vi "Post-Install Custom Action.vi"(10 "Variant":variant) -> (0 "error out":errorcluster)   [LabVIEW 2015]
panel:
  out "Status":string
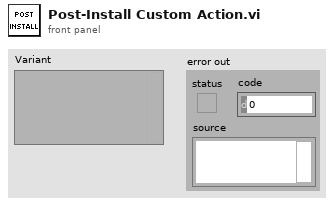
[diagram p1: front panel]
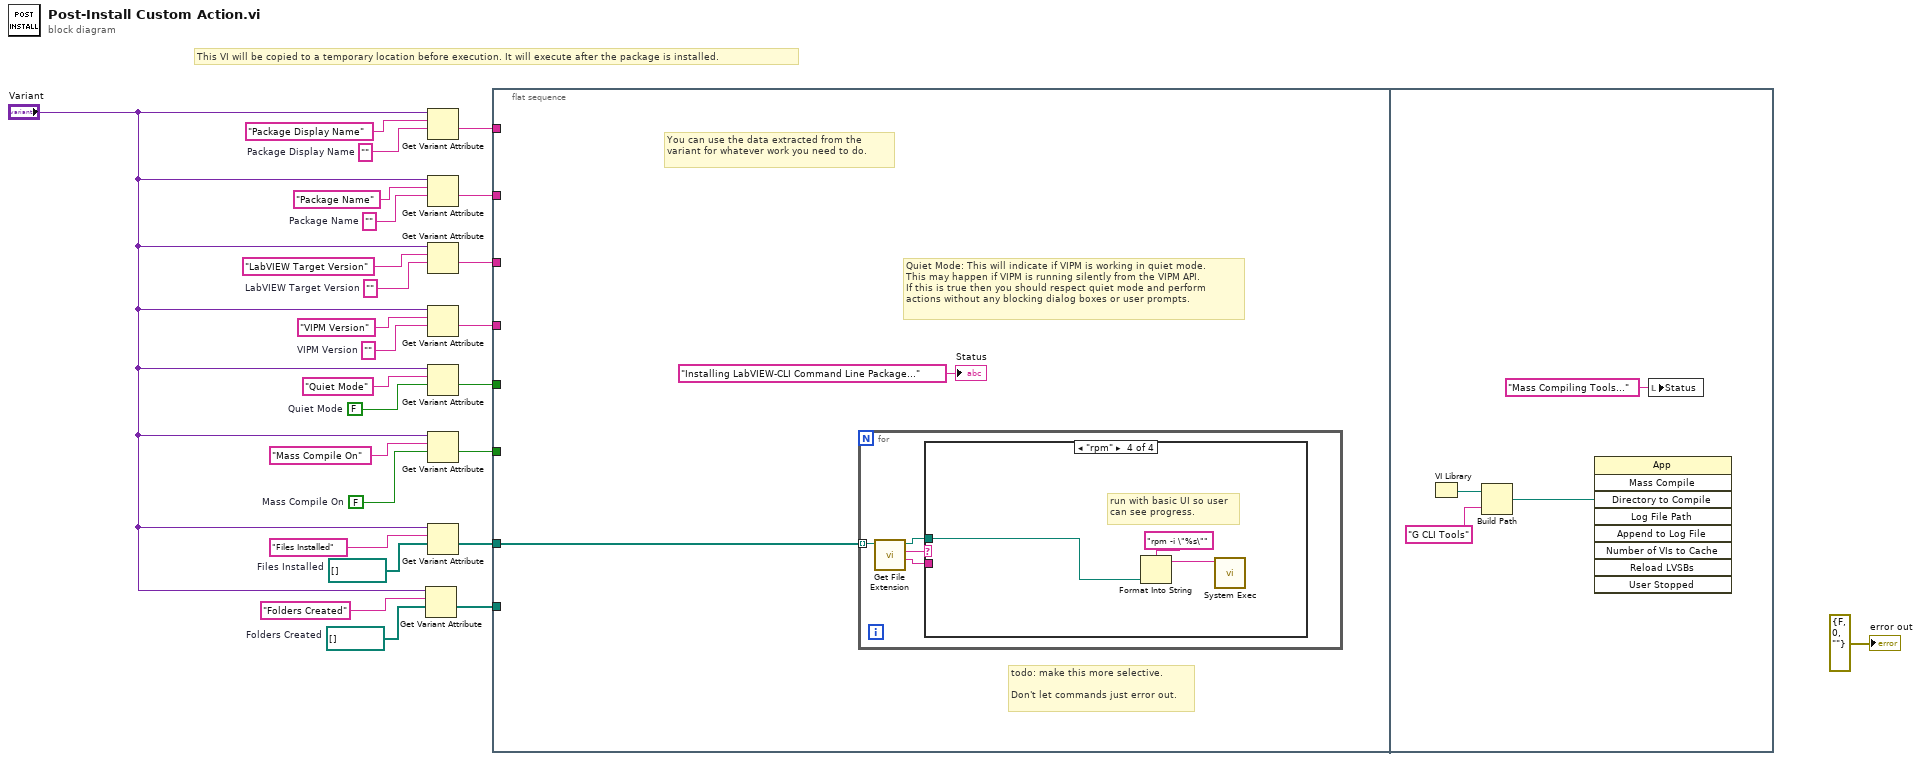
[diagram p0: block diagram]
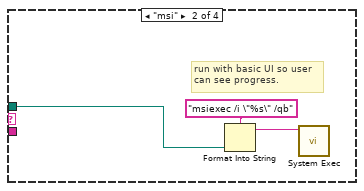
[diagram p3: hidden frame]
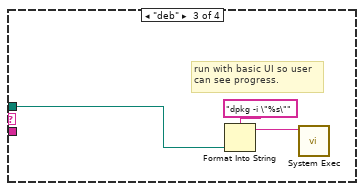
[diagram p4: hidden frame]
diagram:
  w1 = path[] []  # Folders Created
  w2 = path[] []  # Files Installed
  w8 = FALSE  # Mass Compile On
  w9 = ""  # Package Display Name
  w16 = FALSE  # Quiet Mode
  w19 = ""  # VIPM Version
  w21 = ""  # LabVIEW Target Version
  w23 = ""  # Package Name
  # "This VI will be copied to a temporary location before execution. It will execute after the package is installed."
  n1 = Get Variant Attribute(Variant="Variant", name="Folders Created", default value (empty Variant)=w1) -> (value=w6:path[])  [unwired: 1 in, 3 out]
  n2 = Get Variant Attribute(Variant="Variant", name="Package Display Name", default value (empty Variant)=w9) -> (value=w15:string)  [unwired: 1 in, 3 out]
  n3 = Get Variant Attribute(Variant="Variant", name="Package Name", default value (empty Variant)=w23) -> (value=w14:string)  [unwired: 1 in, 3 out]
  n4 = Get Variant Attribute(Variant="Variant", name="LabVIEW Target Version", default value (empty Variant)=w21) -> (value=w13:string)  [unwired: 1 in, 3 out]
  n5 = Get Variant Attribute(Variant="Variant", name="VIPM Version", default value (empty Variant)=w19) -> (value=w12:string)  [unwired: 1 in, 3 out]
  n6 = Get Variant Attribute(Variant="Variant", name="Quiet Mode", default value (empty Variant)=w16) -> (value=w11:bool)  [unwired: 1 in, 3 out]
  n7 = Get Variant Attribute(Variant="Variant", name="Mass Compile On", default value (empty Variant)=w8) -> (value=w10:bool)  [unwired: 1 in, 3 out]
  n8 = Get Variant Attribute(Variant="Variant", name="Files Installed", default value (empty Variant)=w2) -> (value=w5:path[])  [unwired: 1 in, 3 out]
  n9 = flat-sequence {
    tunnel: w15 -> [_]
    tunnel: w14 -> [_]
    tunnel: w13 -> [_]
    tunnel: w12 -> [_]
    tunnel: w11 -> [_]
    tunnel: w10 -> [_]
    tunnel: w5 -> [w28]
    tunnel: w6 -> [_]
    frame #0 {
      # "todo: make this more selective.\n\nDon't let commands just error out."
      # "Quiet Mode: This will indicate if VIPM is working in quiet mode.\nThis may happen if VIPM is running silently from the VIPM API.\nIf this is true then you should respect quiet mode and perform\nactions without any blocking dialog boxes or user prompts."
      # "You can use the data extracted from the variant for whatever work you need to do."
      n10 = for {
        tunnel: w28 -> [w32] mode=indexing
        n11 = call <vilib>:"Get File Extension.vi"("file"=w32) -> ("filename without extension"=w29:string, "lowercase file extension"=w31:string, "dup file"=w30:path)  [unwired: 6 in, 2 out]
        n12 = case shown="\"rpm\"" w31 {
          tunnel: w30 -> [_ w35 w38 w41]
          tunnel: w29 -> [_ _ _ _]
          frame Default {
            # "Not an installer - ignore."
          }
          frame "msi" {
            # "run with basic UI so user\ncan see progress."
            n13 = Format Into String(format string="msiexec /i \"%s\" /qb", w35) -> (resulting string=w33:string)  [unwired: 2 in, 1 out]
            n14 = call <vilib>:"System Exec.vi"("command line"=w33) -> ()  [unwired: 7 in, 4 out]
          }
          frame "deb" {
            # "run with basic UI so user\ncan see progress."
            n15 = Format Into String(format string="dpkg -i \"%s\"", w38) -> (resulting string=w36:string)  [unwired: 2 in, 1 out]
            n16 = call <vilib>:"System Exec.vi"("command line"=w36) -> ()  [unwired: 7 in, 4 out]
          }
          frame "rpm" {
            # "run with basic UI so user\ncan see progress."
            n17 = Format Into String(format string="rpm -i \"%s\"", w41) -> (resulting string=w39:string)  [unwired: 2 in, 1 out]
            n18 = call <vilib>:"System Exec.vi"("command line"=w39) -> ()  [unwired: 7 in, 4 out]
          }
        }
      }
      "Status" <- "Installing LabVIEW-CLI Command Line Package..." ("Status")
    }
    frame #1 {
      n19 = VI Library() -> (path=w45:path)
      n20 = Build Path(base path=w45, name or relative path="G CLI Tools") -> (appended path=w43:path)
      n21 = invoke class="App" method="Mass Compile"("Directory to Compile"=w43) -> ()  [unwired: 8 in, 9 out]
      n22 = local write "Status"("Mass Compiling Tools..." ("Status")) -> ()
    }
  }
  "error out" <- errorcluster {"status"=FALSE, "code"=0, "source"=""} ("error out")
